vi "Finish Tool Call Response.vi"(8 "error in":errorcluster, 9 "server id":i32, 10 "message json":string, 11 "response":string) -> (0 "error out":errorcluster, 3 "response out":string)   [LabVIEW 2020, in "MCP Server.lvlib"]
doc: "Gives the answer of tools/call the form MCP asks for when the call failed.\n\nresponse is what tool call.vi built. If it is not an error it is passed through. If it is an error:\n- the tool name is missing, the tool is not registered, or arguments is not a JSON object: a JSON-RPC error with code -32602 and a short message (a protocol error).\n- anything else (the tool VI is not executable, calling it failed): a normal result with isError true and one text item with the cleaned LabVIEW error message, so that the model can see it and react (a tool execution error).\n\nNo LabVIEW call chain leaves the server."
uses:
  MCP Server.lvlib
  d229d434-7577-429e-aaf5-6b333b1ae36b.vi
  e1c90d8f-b8d7-4728-9011-b5bd1ccec020.vi
  ce3c7441-01fb-487f-bc6d-f81c43e816bc.vi
  add3b3ec-49b5-4a88-8063-6fba70e1b069.vi
  <vilib>/JDP Science/JSONtext/Next JSON Value.vi
  <vilib>/JDP Science/JSONtext/String Subset.vi
  <vilib>/JDP Science/JSONtext/Parsing/Advance past next JSON Value (inlined COPY).vi
  <vilib>/JDP Science/JSONtext/Parsing/Advance past whitespace.vi
  <vilib>/JDP Science/JSONtext/Parsing/Advance past String.vi
  <vilib>/JDP Science/JSONtext/Parsing/Advance past Number.vi
  <vilib>/JDP Science/JSONtext/Parsing/Advance past Line Ending.vi
  <vilib>/JDP Science/JSONtext/Parsing/Parse Full Path or Item Name.vi
  <vilib>/JDP Science/JSONtext/Parsing/Advance past Array.vi
  <vilib>/JDP Science/JSONtext/Parsing/Advance past Object.vi
  <vilib>/JDP Science/JSONtext/support/Error Cluster From Code.vi
  <vilib>/JDP Science/JSONtext/Offset/Find Item Locations by Path.vi
  <vilib>/JDP Science/JSONtext/JSON text to Variant.vi
  <vilib>/JDP Science/JSONtext/Variant to JSON Text.vi
  <vilib>/JDP Science/JSONtext/LVClass Serializer/JSONtext LVClass Serializer.lvclass
  <vilib>/JDP Science/JSONtext/JSONtext.lvlib
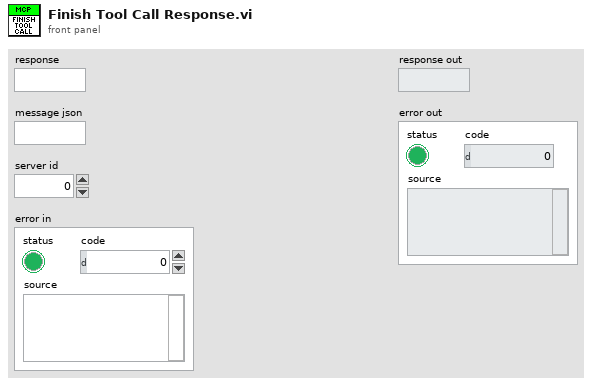
[diagram p1: front panel]
types:
  T1 = typedef "JSONtext.lvlib/JSON Value Type.ctl" = enum16{"Not a JSON Value", "JSON Object", "JSON Array", "String", "Number", "true", "false", "null"}
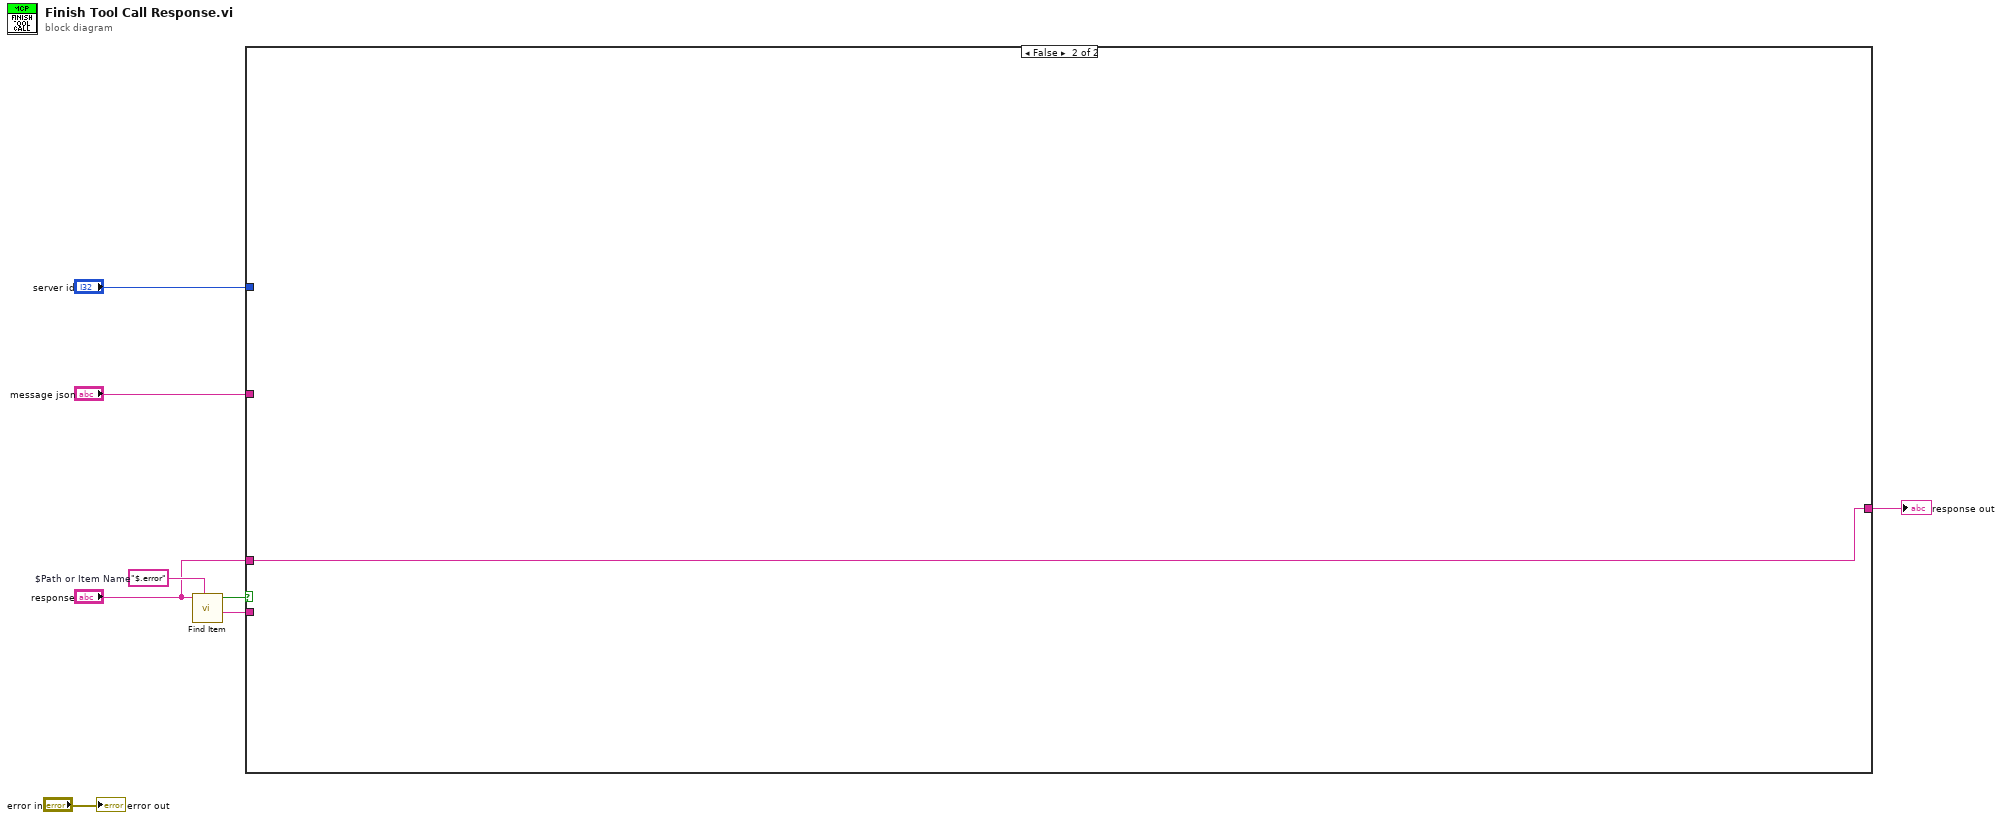
[diagram p0: block diagram]
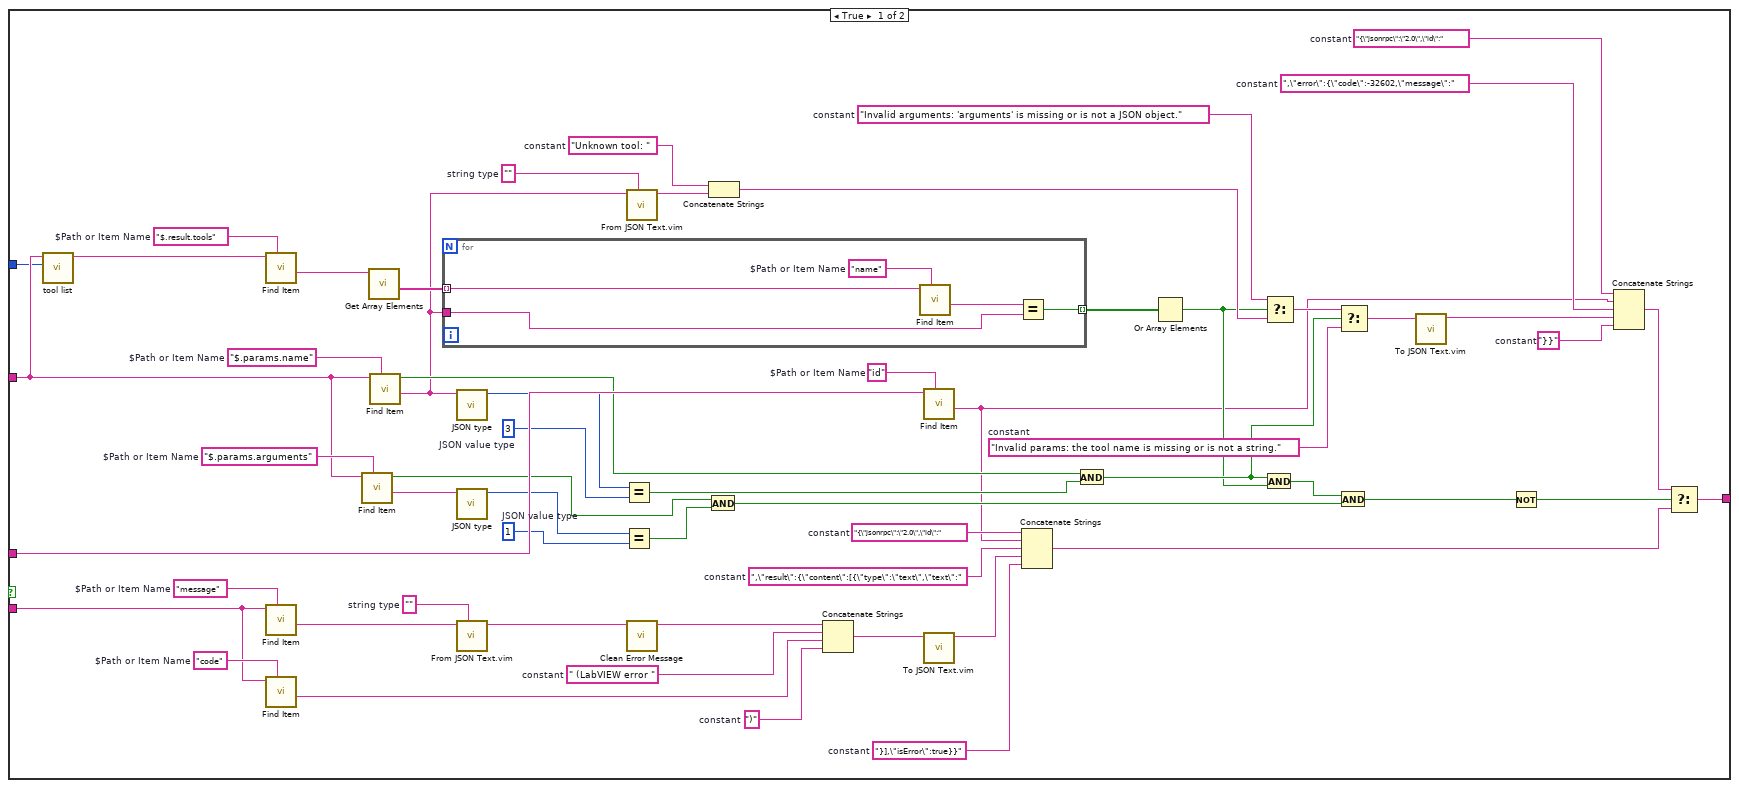
[diagram p2: hidden frame]
diagram:
  w8 = "$.error"  # $Path or Item Name
  n1 = call <vilib>:"Find Item.vi"("$Path or Item Name"=w8, "JSON"="response") -> ("<JSON>"=w6:string, "Found"=w3:bool)  [unwired: 6 in, 2 out]
  n2 = case shown="False" w3 {
    tunnel: "response" -> [w60 w72]
    tunnel: w6 -> [w65 _]
    tunnel: "message json" -> [w47 _]
    tunnel: "server id" -> [w46 _]
    tunnel: [w9 w72] -> w2
    frame True {
      w13 = "}],\"isError\":true}}"  # constant
      w15 = ",\"result\":{\"content\":[{\"type\":\"text\",\"text\":"  # constant
      w17 = "{\"jsonrpc\":\"2.0\",\"id\":"  # constant
      w19 = ")"  # constant
      w21 = " (LabVIEW error "  # constant
      w23 = "}}"  # constant
      w25 = ",\"error\":{\"code\":-32602,\"message\":"  # constant
      w26 = "{\"jsonrpc\":\"2.0\",\"id\":"  # constant
      w33 = "Invalid params: the tool name is missing or is not a string."  # constant
      w36 = "Invalid arguments: 'arguments' is missing or is not a JSON object."  # constant
      w38 = "Unknown tool: "  # constant
      w39 = ""  # string type
      w44 = "$.result.tools"  # $Path or Item Name
      w50 = u16 1  # JSON value type
      w53 = "$.params.arguments"  # $Path or Item Name
      w56 = u16 3  # JSON value type
      w58 = "$.params.name"  # $Path or Item Name
      w59 = "id"  # $Path or Item Name
      w62 = ""  # string type
      w64 = "message"  # $Path or Item Name
      w66 = "code"  # $Path or Item Name
      n3 = call "tool list.vi"("server id in"=w46, "message json"=w47) -> ("response"=w45:string)  [unwired: 8 in, 1 out]
      n4 = call <vilib>:"Find Item.vi"("$Path or Item Name"=w44, "JSON"=w45) -> ("<JSON>"=w43:string)  [unwired: 6 in, 3 out]
      n5 = call <vilib>:"Find Item.vi"("$Path or Item Name"=w64, "JSON"=w65) -> ("<JSON>"=w63:string)  [unwired: 6 in, 3 out]
      n6 = call <vilib>:"Find Item.vi"("$Path or Item Name"=w66, "JSON"=w65) -> ("<JSON>"=w20:string)  [unwired: 6 in, 3 out]
      n7 = call <vilib>:"Find Item.vi"("$Path or Item Name"=w53, "JSON"=w47) -> ("<JSON>"=w52:string, "Found"=w49:bool)  [unwired: 6 in, 2 out]
      n8 = call <vilib>:"Get Array Elements.vi"("JSON"=w43) -> ("<JSON>"=w42:string[])  [unwired: 8 in, 2 out]
      n9 = call <vilib>:"Find Item.vi"("$Path or Item Name"=w58, "JSON"=w47) -> ("<JSON>"=w40:string, "Found"=w55:bool)  [unwired: 6 in, 2 out]
      n10 = for {
        tunnel: w42 -> [w71] mode=indexing
        tunnel: w40 -> [w68]
        tunnel: [w67] -> w41 mode=indexing
        w70 = "name"  # $Path or Item Name
        n11 = call <vilib>:"Find Item.vi"("$Path or Item Name"=w70, "JSON"=w71) -> ("<JSON>"=w69:string)  [unwired: 6 in, 3 out]
        n12 = Equal?(x=w69, y=w68) -> (x = y?=w67:bool)
      }
      n13 = call <vilib>:"JSON type.vi"("JSON"=w40) -> ("JSON Value Type"=w57:T1)  [unwired: 9 in, 1 out]
      n14 = call <vilib>:"JSON type.vi"("JSON"=w52) -> ("JSON Value Type"=w51:T1)  [unwired: 9 in, 1 out]
      n15 = call "From JSON Text.vim"("Data Type and Default Value"=w62, "JSON"=w63) -> ("Data out"=w61:string)  [unwired: 8 in, 1 out]
      n16 = Equal?(x=w57, y=w56) -> (x = y?=w54:bool)
      n17 = Equal?(x=w51, y=w50) -> (x = y?=w48:bool)
      n18 = call "From JSON Text.vim"("Data Type and Default Value"=w39, "JSON"=w40) -> ("Data out"=w37:string)  [unwired: 8 in, 1 out]
      n19 = call "Clean Error Message.vi"("source"=w61) -> ("message"=w22:string)  [unwired: 10 in]
      n20 = And(x=w49, y=w48) -> (x .and. y?=w29:bool)
      n21 = Concatenate Strings(w38, w37) -> (w35:string)
      n22 = Concatenate Strings(w22, w21, w20, w19) -> (w18:string)
      n23 = call <vilib>:"Find Item.vi"("$Path or Item Name"=w59, "JSON"=w60) -> ("<JSON>"=w16:string)  [unwired: 6 in, 3 out]
      n24 = call "To JSON Text.vim"("Anything"=w18) -> ("<JSON>"=w14:string)  [unwired: 9 in, 1 out]
      n25 = Concatenate Strings(w17, w16, w15, w14, w13) -> (w10:string)
      n26 = And(x=w55, y=w54) -> (x .and. y?=w32:bool)
      n27 = Or Array Elements(Boolean array=w41) -> (logical OR=w31:bool)
      n28 = And(x=w32, y=w31) -> (x .and. y?=w30:bool)
      n29 = Select(t=w36, s=w31, f=w35) -> (s? t:f=w34:string)
      n30 = And(x=w30, y=w29) -> (x .and. y?=w28:bool)
      n31 = Select(t=w34, s=w32, f=w33) -> (s? t:f=w27:string)
      n32 = call "To JSON Text.vim"("Anything"=w27) -> ("<JSON>"=w24:string)  [unwired: 9 in, 1 out]
      n33 = Not(x=w28) -> (.not. x?=w11:bool)
      n34 = Concatenate Strings(w26, w16, w25, w24, w23) -> (w12:string)
      n35 = Select(t=w12, s=w11, f=w10) -> (s? t:f=w9:string)
    }
    frame False {
    }
  }
  "response out" <- w2
  "error out" <- "error in"
